vi "Assert Almost Equal_Float.vi"(3 "Execution time (s)":dbl=-1.0, 4 "Use Percentage of X (F)":bool, 5 "Assert Only? (F)":bool, 6 "error code (1)":i32=1, 7 "Label":string, 8 "error in (no error)":errorcluster, 9 "Tolerance":ext=0.00000100000000000000000004, 10 "Actual":ext, 11 "Expected":ext) -> (0 "error out":errorcluster, 2 "Properties.Assert":refnum<class "Properties.Assert.lvclass">)   [LabVIEW 2013, in "Caraya.lvlib" / "Assert.lvclass"]
doc: "Generates an error if the input condition is not met.\n\nTolerance is either an absolute or percentage value, depending on the \"Use Percentage of X\" flag. Defaults to absolute, tolerance = 1E-6.\nWhen Percentage mode, percentage is calculated based on value of X.\n\n\n--\nCopyright © 2015 JKI All rights reserved.\n\nAuthor: Tomi Maila <tomi.maila@jki.net>\n\nThis library is provided \"AS IS\" ,WITHOUT WARRANTIES OR\nCONDITIONS OF ANY KIND, either express or implied.\n\nJKI -- jki.net"
uses:
  Assert.lvclass
  Properties.Assert/Properties.Assert.lvclass
  Properties/Properties.lvclass
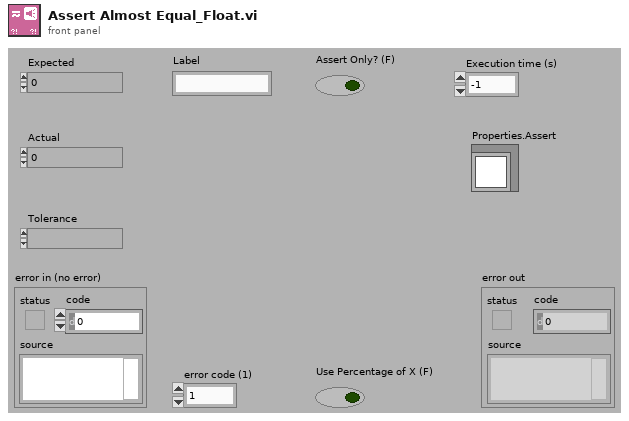
[diagram p1: front panel]
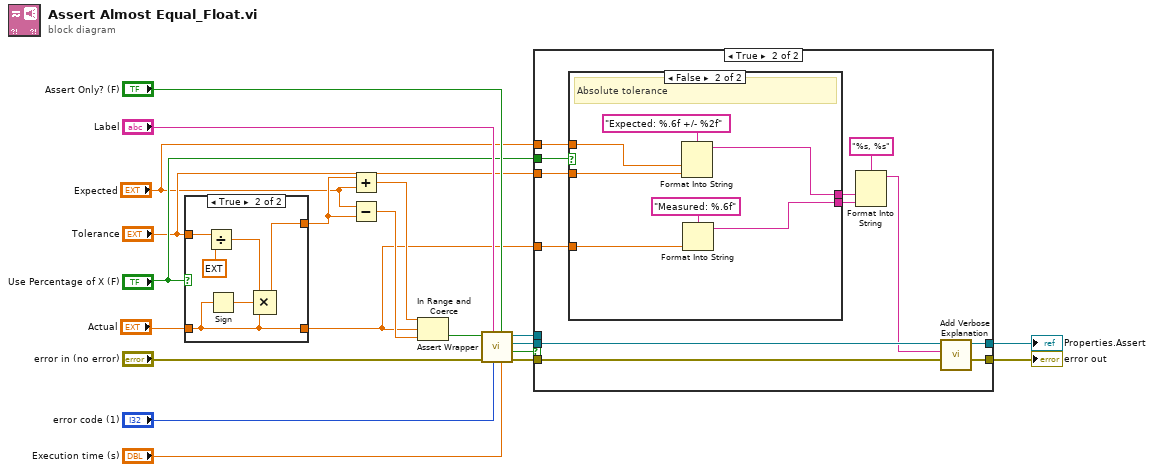
[diagram p0: block diagram]
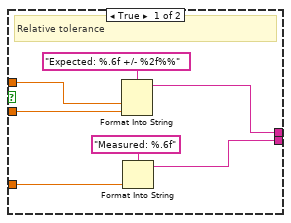
[diagram p3: hidden frame]
diagram:
  n1 = case shown="True" "Use Percentage of X (F)" {
    tunnel: "Tolerance" -> [w22 w28]
    tunnel: [w22 w25] -> w14
    tunnel: "Actual" -> [w21 w24]
    tunnel: [w21 w24] -> w10
    frame False {
    }
    frame True {
      n2 = Divide(x=w28, y=ext 100.0) -> (x/y=w23:ext)
      n3 = Sign(1:w24) -> (0:w26:ext)
      n4 = Compound Arithmetic op=MULTIPLY(w23, w26, w24) -> (w25:ext)
    }
  }
  n5 = Add(x=w14, y="Expected") -> (x+y=w16:ext)
  n6 = Subtract(x="Expected", y=w14) -> (x-y=w15:ext)
  n7 = In Range and Coerce(upper limit=w16, x=w10, lower limit=w15) -> (In Range?=w17:bool)  [unwired: 1 out]
  n8 = call "Assert Wrapper.vi"("Execution time (s)"="Execution time (s)", "Assert Only? (F)"="Assert Only? (F)", "error code (1)"="error code (1)", "Label"="Label", "error in (no error)"="error in (no error)", "Assert?"=w17) -> ("error out"=w6:errorcluster, "Verbose"=w7:bool, "Properties.Assert"=w4:refnum<class "Properties.Assert.lvclass">, "Assert out"=w5:refnum<class "Assert.lvclass">)  [unwired: 2 in]
  n9 = case shown="True" w7 {
    tunnel: [w30 w32] -> w12
    tunnel: w5 -> [_ _]
    tunnel: w6 -> [w30 w33]
    tunnel: "Use Percentage of X (F)" -> [_ w39]
    tunnel: "Expected" -> [_ w38]
    tunnel: w10 -> [_ w37]
    tunnel: "Tolerance" -> [_ w36]
    tunnel: w4 -> [w29 w35]
    tunnel: [w29 w31] -> w3
    frame False {
    }
    frame True {
      n10 = case shown="False" w39 {
        tunnel: [w48 w55] -> w41
        tunnel: [w46 w53] -> w40
        tunnel: w38 -> [w44 w51]
        tunnel: w37 -> [w45 w52]
        tunnel: w36 -> [w43 w50]
        frame True {
          # "Relative tolerance"
          n11 = Format Into String(format string="Expected: %.6f +/- %2f%%", w44, w43) -> (resulting string=w48:string)  [unwired: 2 in, 1 out]
          n12 = Format Into String(format string="Measured: %.6f", w45) -> (resulting string=w46:string)  [unwired: 2 in, 1 out]
        }
        frame False {
          # "Absolute tolerance"
          n13 = Format Into String(format string="Expected: %.6f +/- %2f", w51, w50) -> (resulting string=w55:string)  [unwired: 2 in, 1 out]
          n14 = Format Into String(format string="Measured: %.6f", w52) -> (resulting string=w53:string)  [unwired: 2 in, 1 out]
        }
      }
      n15 = Format Into String(format string="%s, %s", w41, w40) -> (resulting string=w34:string)  [unwired: 2 in, 1 out]
      n16 = call "Add Verbose Explanation.vi"("error in (no error)"=w33, "Verbose Explanation"=w34, "Properties"=w35) -> ("error out"=w32:errorcluster, "Properties"=w31:refnum<class "Properties.Assert.lvclass">)  [unwired: 7 in]
    }
  }
  "error out" <- w12
  "Properties.Assert" <- w3
